vi "Result_Resolve_Reference.vi"(8 "error in (no error)":errorcluster={"status"=FALSE, "code"=0, "source"="\"\""}, 10 "reference key":string, 11 "Current run/step/cycle IDs":string) -> (0 "error out":errorcluster={"status"=FALSE, "code"=0, "source"="\"\""}, 2 "status ok":bool, 3 "Typed stored result":string)   [LabVIEW 2026]
doc: "INTENT: Fetch earlier stored measurement. LOGIC: Resolve named historical result with permitted scope and immutable identity."
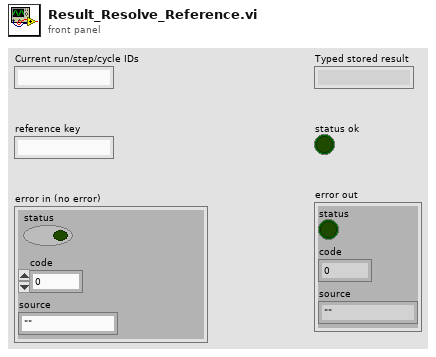
[diagram p1: front panel]
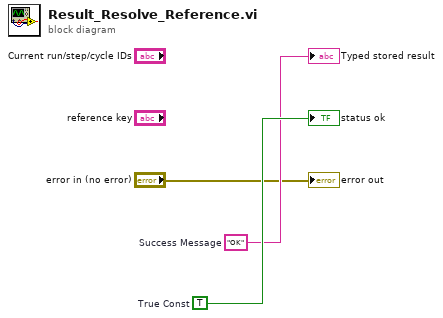
[diagram p0: block diagram]
diagram:
  w3 = TRUE  # True Const
  w2 = "OK"  # Success Message
  "Typed stored result" <- w2
  "status ok" <- w3
  "error out" <- "error in (no error)"
